vi "set NR HO UL_DL Channel BandWidth.vi"(8 "error in (no error)":errorcluster caption="에러 입력(에러 없음)", 9 "Direction":T1, 10 "Bandwidth Setting Param":T2, 11 "Anritsu Call Box_Implement 입력":refnum<class "Anritsu Call Box_Implement.lvclass">) -> (0 "error out":errorcluster caption="에러 출력", 3 "Anritsu Call Box_Implement 출력":refnum<class "Anritsu Call Box_Implement.lvclass">)   [LabVIEW 2023, in "ANRITSU Call Box.lvlib" / "Anritsu Call Box_Implement.lvclass"]
uses:
  Anritsu Call Box_Implement.lvclass
  Anritsu Call Box_Implement.lvclass/Anritsu Call Box_Implement.ctl
  NR/NR.lvclass
  Type Definition/NR Channel Bandwidth Param.ctl
  ANRITSU Call Box.lvlib
  Type Definition/Uplink Downlink Enum.ctl
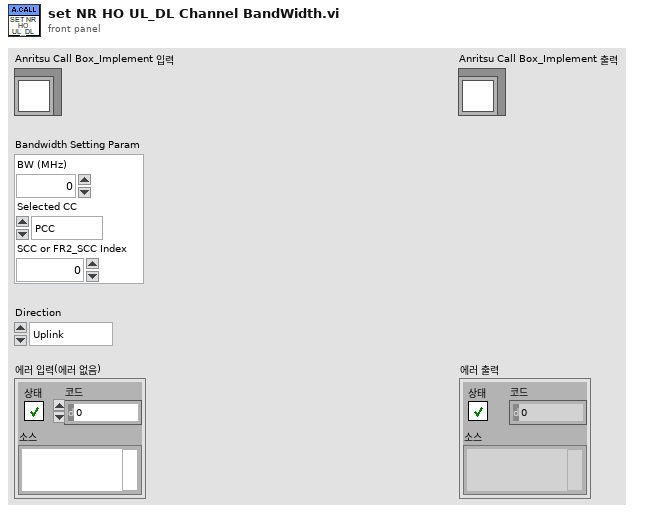
[diagram p1: front panel]
types:
  T1 = typedef "ANRITSU Call Box.lvlib/Uplink Downlink Enum.ctl" = enum16{"Uplink", "Downlink"}
  T2 = typedef "ANRITSU Call Box.lvlib/NR Channel Bandwidth Param.ctl" = cluster{"BW (MHz)":u32, "Selected CC":enum16{"PCC", "SCC", "FR2_PCC", "FR2_SCC"}, "SCC or FR2_SCC Index":u32}
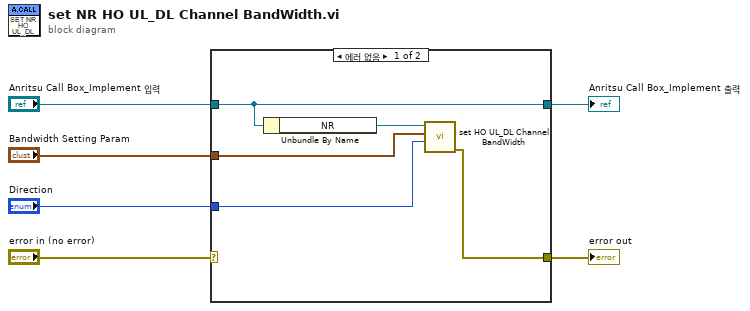
[diagram p0: block diagram]
diagram:
  n1 = case shown="에러 없음" "error in (no error)" {
    selector: "error in (no error)" -> [_ w12]
    tunnel: "Anritsu Call Box_Implement 입력" -> [w11 w13]
    tunnel: [w11 w13] -> w4
    tunnel: [w7 w12] -> w3
    tunnel: "Bandwidth Setting Param" -> [w9 _]
    tunnel: "Direction" -> [w8 _]
    frame No Error {
      n2 = Unbundle By Name(w11) -> ("NR"=w10:refnum<class "NR.lvclass">)
      n3 = call "set HO UL_DL Channel BandWidth.vi"("Direction"=w8, "Bandwidth Setting Param"=w9, "NR 입력"=w10) -> ("error out"=w7:errorcluster)  [unwired: 7 in, 1 out]
    }
    frame Error {
    }
  }
  "error out" <- w3
  "Anritsu Call Box_Implement 출력" <- w4
